vi "CIVI Close.vi"(8 "error in":errorcluster, 11 "VISA Session in":refnum<visa-resource-name>) -> (0 "error out":errorcluster)   [LabVIEW 2026]
doc: "Closes the VISA session using VISA Close.\nAccepts an upstream error so cleanup can still run.\nReturns the error status from VISA Close."
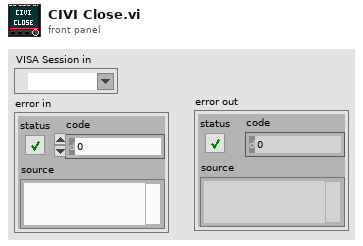
[diagram p1: front panel]
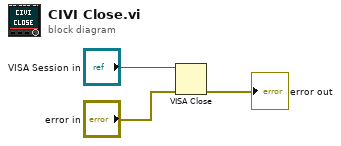
[diagram p0: block diagram]
diagram:
  n1 = VISA Close(VISA resource name="VISA Session in", error in (no error)="error in") -> (error out=→"error out":errorcluster)
